vi "Get Handle.vi"(8 "error in (no error)":errorcluster, 10 "PID":u32, 11 "VID":u32) -> (0 "error out":errorcluster, 2 "HANDLE":u32)   [LabVIEW 2017, in "HID_ARZ.lvlib"]
uses:
  HID_ARZ.lvlib
  <userlib>/HID_ARZ/mcHID.dll
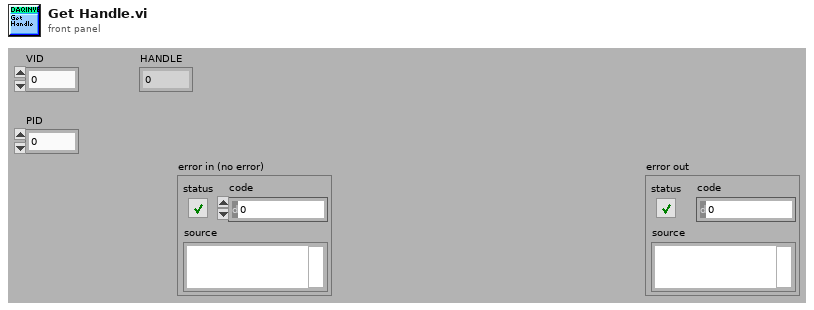
[diagram p1: front panel]
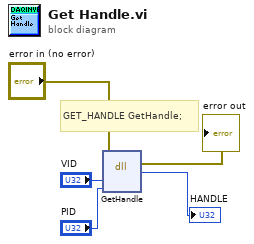
[diagram p0: block diagram]
diagram:
  # "GET_HANDLE GetHandle;"
  n1 = dll-call lib="C:/Program Files (x86)/National Instruments/LabVIEW 2017/user.lib/HID_ARZ/mcHID.dll" fn="GetHandle"(error in="error in (no error)", "VID"="VID", "PID"="PID") -> (error out=→"error out":errorcluster, "HANDLE"=→"HANDLE":u32)  [unwired: 4 in, 1 out]
